vi "GDSLvClass_ReadClassColors.vi"(0 "Library Refnum":refnum<vi>, 2 "OnlyReadClassItemIcon(False)":bool, 5 "error in (no error)":errorcluster) -> (14 "Library Refnum":refnum<vi>, 15 "LvClassIconSettings":T2={"Frame"=0, "Frame thickness"=3, "Header Background"=8453954, "Header Text"=0, "ColorPublic"=16121600, "ColorProtected"=16777215, "ColorPrivate"=16777215, "Body Text"=0, "ClassBodyIcon"=""} {"Frame thickness" min=1 max=3 step=1}, 16 "LvClassIconSettingsFound":bool, 17 "ClassItemIconName(NoExtension)":string, 18 "Type":T1=enum."Library", 19 "error out":errorcluster)   [LabVIEW 2020]
uses:
  <resource>/Framework/Providers/Open_GDS/ClassProviders/Common/LvClass_class/GDSLvClass_IconSettingsType.ctl
  <resource>/Framework/Providers/Open_GDS/ClassProviders/Common/LvIcon_class/GDSLvIcon_Type.ctl
  <resource>/Framework/Providers/Open_GDS/SubVIs/GOOP_ClassSettingsMemory_Action.ctl
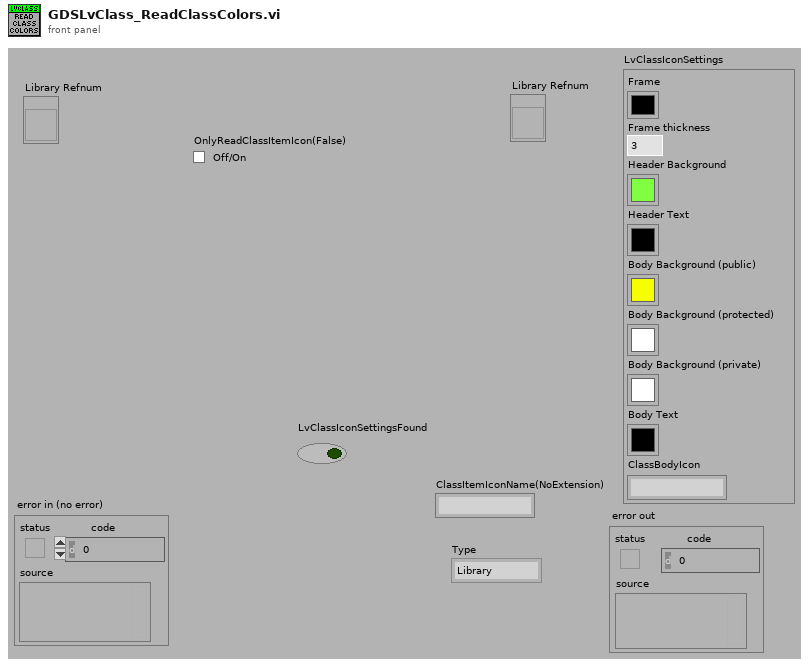
[diagram p1: front panel]
types:
  T1 = typedef "GDSLvIcon_Type.ctl" = enum16{"LvClass", "Library", "X-Control", "LvInterface"}
  T2 = typedef "GDSLvClass_IconSettingsType.ctl" = cluster{"Frame":u32, "Frame thickness":u8, "Header Background":u32, "Header Text":u32, "ColorPublic":u32, "ColorProtected":u32, "ColorPrivate":u32, "Body Text":u32, "ClassBodyIcon":string}
  T3 = typedef "GOOP_ClassSettingsMemory_Action.ctl" = enum16{"Read", "Write", "Read (ClassItemIconOnly)"}
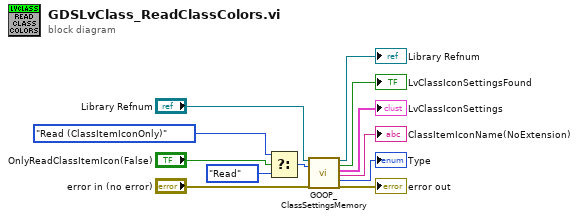
[diagram p0: block diagram]
diagram:
  n1 = Select(t=GOOP_ClassSettingsMemory_Action."Read (ClassItemIconOnly)", s="OnlyReadClassItemIcon(False)", f=GOOP_ClassSettingsMemory_Action."Read" ("Action")) -> (s? t:f=w2:T3)
  n2 = call <resource>:"GOOP_ClassSettingsMemory.vi"("Library Refnum"="Library Refnum", "Action"=w2, "error in"="error in (no error)") -> ("Library Refnum"=→"Library Refnum":refnum<vi>, "Found"=→"LvClassIconSettingsFound":bool, "LvClassIconSettings"=→"LvClassIconSettings":T2, "ItemIcon"=→"ClassItemIconName(NoExtension)":string, "Type"=→"Type":T1, "error out"=→"error out":errorcluster)  [unwired: 11 in]
